vi "Set Name.vi"(8 "error in":errorcluster, 10 "Name":string, 11 "Element in":refnum<class "Element.lvclass">) -> (0 "error out":errorcluster, 3 "Element out":refnum<class "Element.lvclass">)   [LabVIEW 2026, in "Element.lvclass"]
doc: "Set Name."
uses:
  Element.lvclass
  Element.lvclass/Element.ctl
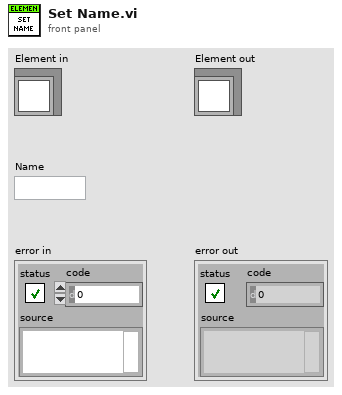
[diagram p1: front panel]
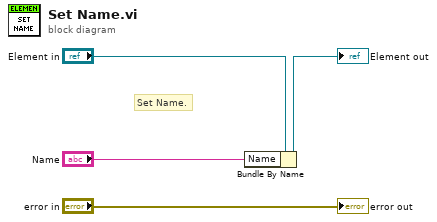
[diagram p0: block diagram]
diagram:
  # "Set Name."
  n1 = Bundle By Name(cluster="Element in", "Name"="Name") -> (→"Element out":refnum<class "Element.lvclass">)
  "error out" <- "error in"
